vi "SubscribeChamberStatusUpdated Send Stream.vi"(6 "Heater State":T1, 8 "Temperature Ramp Rate":dbl, 9 "Temperature Set Point":dbl, 10 "Actual Temperature":dbl, 11 "input cluster":T2={"gRPCid"=0, "Active"=FALSE, "timeout"=-1}) -> (0 "error out":errorcluster)   [LabVIEW 2020]
doc: "Send data with <b>Streaming?</b> parameter set to True to maintain stream active."
uses:
  Stream Data--cluster.ctl
  <vilib>/gRPC/LabVIEW gRPC Library/Shared/grpcId.ctl
  Program Files (x86)/National Instruments/LabVIEW 2020/examples/DQMH Consortium/DQMH Fundamentals - Thermal Chamber/Libraries/Thermal Chamber Controller_DQMH/Heater State--enum.ctl
  thermal-chamber-controller_server/RPC Messages/lv_python_grpc_webui_demo_v1_ChamberStatus.ctl
  thermal-chamber-controller_server/RPC Messages/lv_python_grpc_webui_demo_v1_HeaterState.ctl
  thermal-chamber-controller_server/thermal-chamber-controller_server.lvlib
  thermal-chamber-controller_server/RPC Service/ThermalChamberController/ThermalChamberController.lvclass
  <vilib>/gRPC/LabVIEW gRPC Library/grpc-lvsupport-release.lvlib
  Program Files (x86)/National Instruments/LabVIEW 2020/examples/DQMH Consortium/DQMH Fundamentals - Thermal Chamber/Libraries/Thermal Chamber Controller_DQMH/Thermal Chamber Controller_DQMH.lvlib
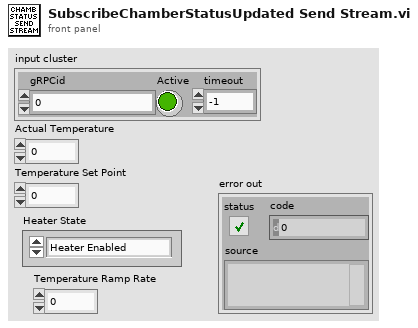
[diagram p1: front panel]
types:
  T1 = typedef "Thermal Chamber Controller_DQMH.lvlib/Heater State--enum.ctl" = enum16{"Heater Enabled", "Heater Disabled"}
  T2 = typedef "Stream Data--cluster.ctl" = cluster{"gRPCid":T3, "Active":bool, "timeout":i32}
  T3 = typedef "grpc-lvsupport-release.lvlib/grpcId.ctl" = u64
  T4 = typedef "thermal-chamber-controller_server.lvlib/lv_python_grpc_webui_demo_v1_ChamberStatus.ctl" = cluster{"actual_temperature":dbl, "temperature_set_point":dbl, "temperature_ramp_rate":dbl, "heater_state":T5}
  T5 = typedef "thermal-chamber-controller_server.lvlib/lv_python_grpc_webui_demo_v1_HeaterState.ctl" = enum32{"HEATER_ENABLED", "HEATER_DISABLED"}
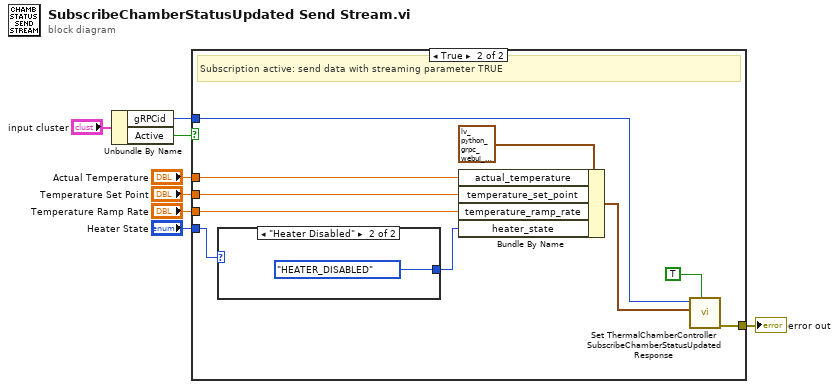
[diagram p0: block diagram]
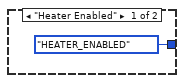
[diagram p3: hidden frame]
diagram:
  n1 = Unbundle By Name("input cluster") -> ("gRPCid"=w8:T3, "Active"=w1:bool)
  n2 = case shown="True" w1 {
    tunnel: "Actual Temperature" -> [_ w17]
    tunnel: "Temperature Set Point" -> [_ w16]
    tunnel: "Temperature Ramp Rate" -> [_ w15]
    tunnel: "Heater State" -> [_ w10]
    tunnel: w8 -> [_ w13]
    tunnel: [_ w12] -> w2
    frame False {
      # "Inactive: no action."
    }
    frame True {
      # "Subscription active: send data with streaming parameter TRUE"
      n3 = case shown="\"Heater Disabled\"" w10 {
        tunnel: [lv_python_grpc_webui_demo_v1_HeaterState."HEATER_ENABLED" ("heater_state") lv_python_grpc_webui_demo_v1_HeaterState."HEATER_DISABLED" ("heater_state")] -> w9
        frame "Heater Enabled" {
        }
        frame "Heater Disabled" {
        }
      }
      n4 = Bundle By Name(cluster=T4 {"actual_temperature"=0.0, "temperature_set_point"=0.0, "temperature_ramp_rate"=0.0, "heater_state"=enum."HEATER_ENABLED"} ("Message Data"), "actual_temperature"=w17, "temperature_set_point"=w16, "temperature_ramp_rate"=w15, "heater_state"=w9) -> (w14:T4)
      n5 = call "Set ThermalChamberController SubscribeChamberStatusUpdated Response.vi"("Streaming? (F)"=TRUE, "Message Data"=w14, "gRPCid in"=w13) -> ("error out"=w12:errorcluster)  [unwired: 8 in]
    }
  }
  "error out" <- w2
